vi "LinearSystemId_CreateFlywheelSystem.vi"(9 "G":dbl, 10 "jKgMetersSquared":dbl, 11 "DCMOTOR":T1 {"Jr_KgM2" format="%13.5p"; "L_H" format="%13.5p"; "Kt_NMPerAmp" format="%13.5p"; "KvINV_RadPerSecPerVolt" format="%13.5p"; "R_Ohms" format="%13.5p"; "FreeSpeed_RadPerSec" format="%13.5p"; "FreeCurrent_Amps" format="%13.5p"; "StallCurrent_Amps" format="%13.5p"; "StallTorque_NM" format="%13.5p"; "nominalVoltage_Volts" format="%13.5p"}) -> (0 "Error":bool, 3 "Linearsystem":T2)   [LabVIEW 2019, in "Trajectory_Library.lvlib"]
doc: "Create a state-space model of a flywheel system. The states of the system are [angular velocity], inputs are [voltage], and outputs are [angular velocity].\n\n\nThe flywheel linear system definition is:\n - States\n - angular velocity (Rad/Sec)\n - Inputs:\n - motor voltage\n - Outputs:\n - angular velocity (rad/sec)\n\n\nInputs: \n - motor -- The motor (or gearbox) attached to the arm.\n - jKgMetersSquared -- The moment of inertia J of the flywheel.\n - G -- The reduction between motor and drum, as a ratio of output to input.\n\nOutputs:\n - LinearSystem -- A LinearSystem representing the given characterized constants.\n - Error -- A boolean indicating an error occured creating the system. A value of TRUE indicates an error."
uses:
  Trajectory_Library.lvlib
  TypeDef/LINEAR_SYSTEM.ctl
  <vilib>/Analysis/Matrix/Datatypes/RealMatrix.ctl
  TypeDef/DCMOTOR.CTL
  MatrixHelper_CoerceSize.vi
  <vilib>/Analysis/7linalg.llb/Create Special Matrix.vi
  <vilib>/Analysis/7linalg.llb/Create Special Real Matrix.vi
  <vilib>/Analysis/Matrix/NI_Matrix.lvlib
panel:
  # "<States,States>"
  # "<States,Inputs>"
  # "<Outputs,States>"
  # "<Outputs,Inputs>"
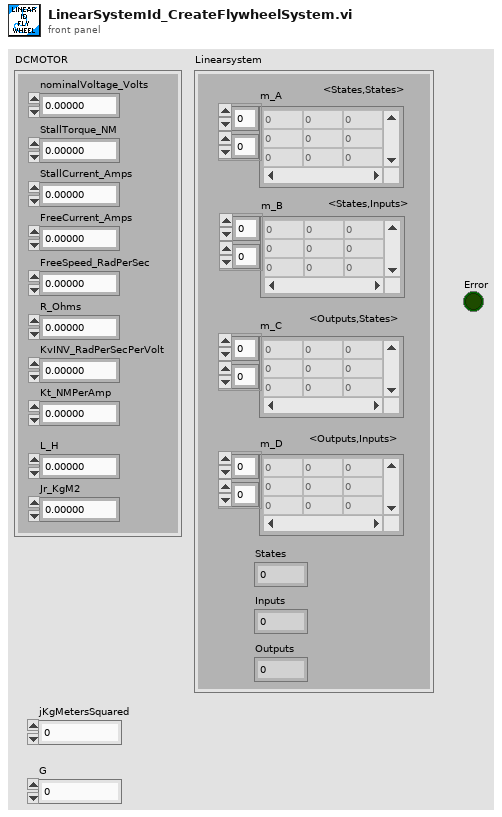
[diagram p1: front panel]
types:
  T1 = typedef "Trajectory_Library.lvlib/DCMOTOR.CTL" = cluster{"nominalVoltage_Volts":dbl, "StallTorque_NM":dbl, "StallCurrent_Amps":dbl, "FreeCurrent_Amps":dbl, "FreeSpeed_RadPerSec":dbl, "R_Ohms":dbl, "KvINV_RadPerSecPerVolt":dbl, "Kt_NMPerAmp":dbl, "L_H":dbl, "Jr_KgM2":dbl}
  T2 = typedef "Trajectory_Library.lvlib/LINEAR_SYSTEM.ctl" = cluster{"m_A":T3, "m_B":T3, "m_C":T3, "m_D":T3, "States":i32, "Inputs":i32, "Outputs":i32}
  T3 = typedef "NI_Matrix.lvlib/RealMatrix.ctl" = dbl[][]
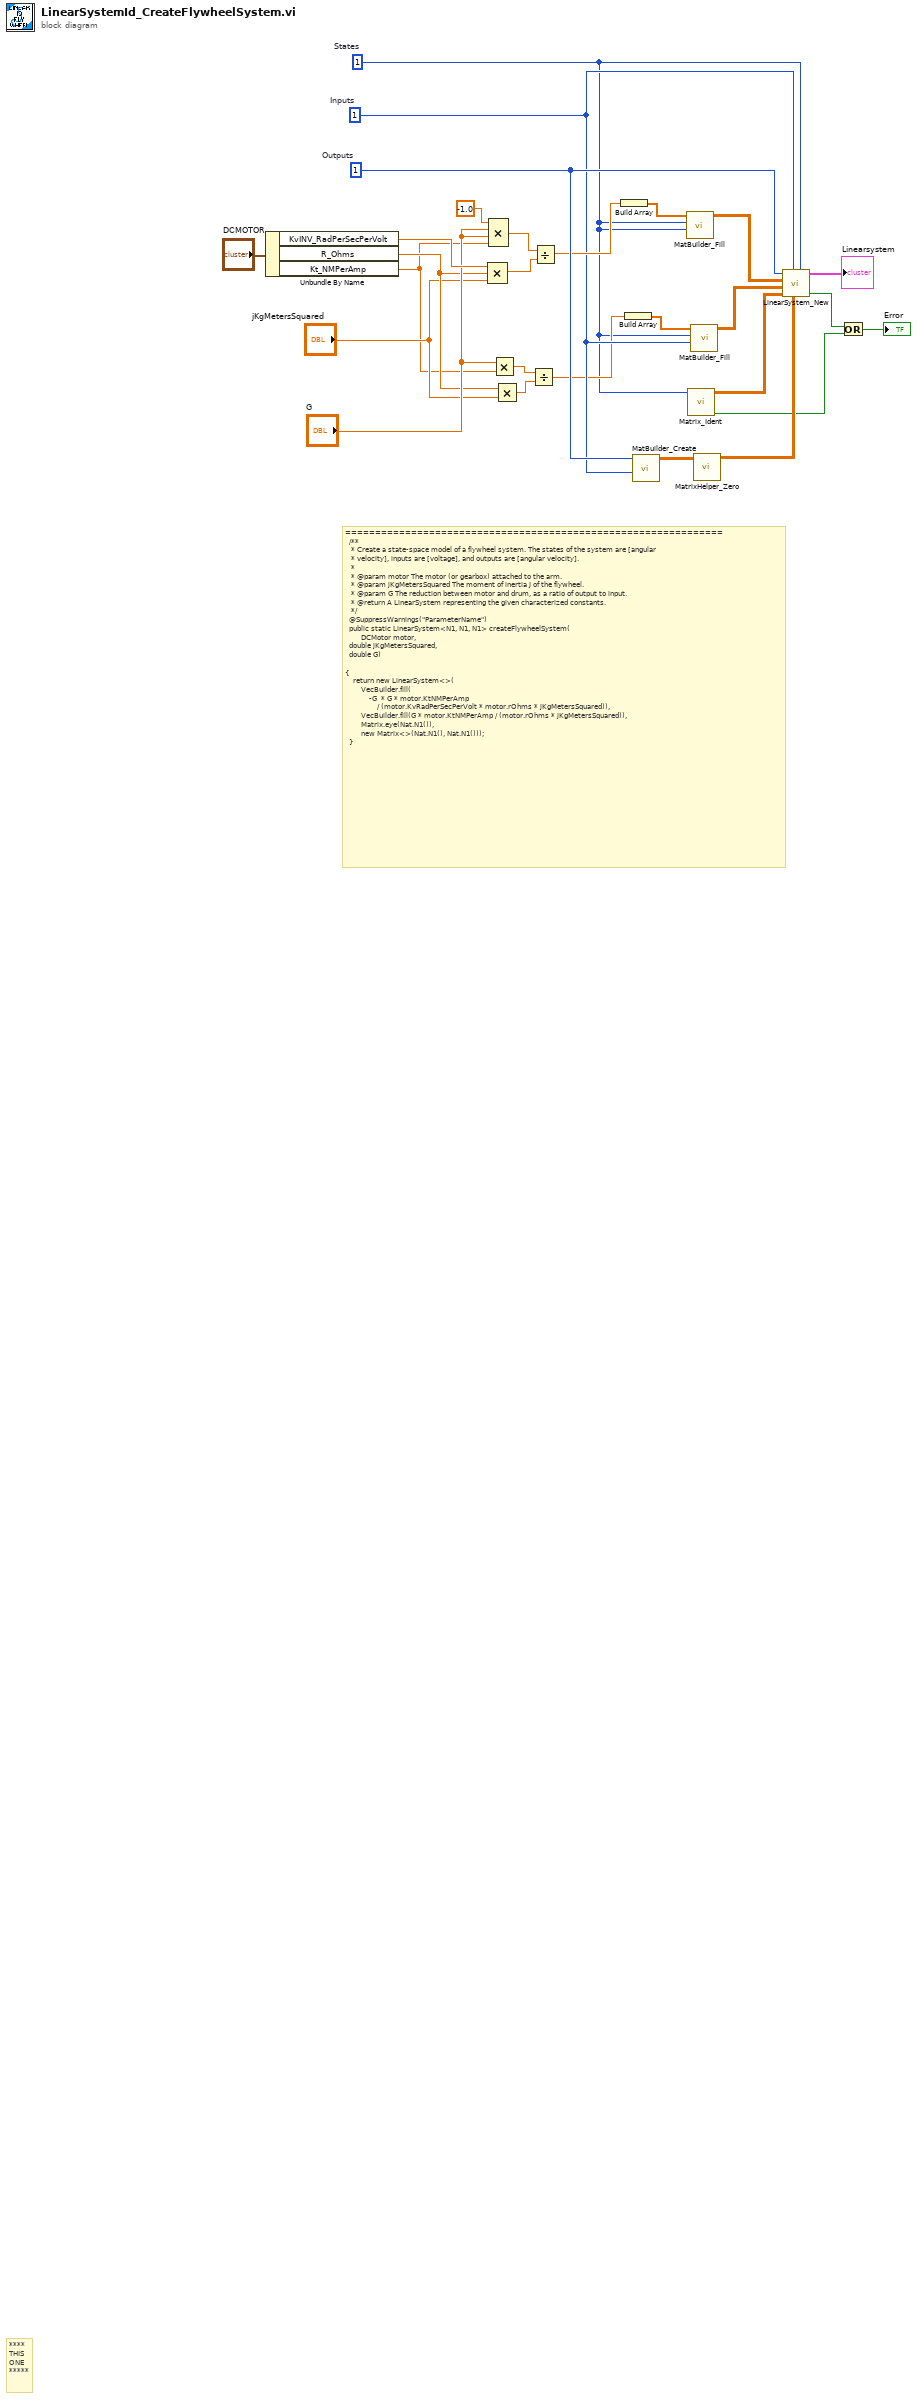
[diagram p0: block diagram]
diagram:
  w5 = 1  # States
  w8 = 1  # Inputs
  w15 = 1  # Outputs
  # "===============================================================\n  /**\n   * Create a state-space model of a flywheel system. The states of the system are [angular\n   * velocity], inputs are [voltage], and outputs are [angular velocity].\n   *\n   * @param motor The motor (or gearbox) attached to the arm.\n   * @param jKgMetersSquared The moment of inertia J of the flywheel.\n   * @param G The reduction between motor and drum, as a ratio of output to input.\n   * @return A LinearSystem representing the given characterized constants.\n   */\n  @SuppressWarnings(\"ParameterName\")\n  public static LinearSystem<N1, N1, N1> createFlywheelSystem(\n      \t\tDCMotor motor, \n\t\tdouble jKgMetersSquared, \n\t\tdouble G) \n\n{\n    return new LinearSystem<>(\n        VecBuilder.fill(\n            -G  * G * motor.KtNMPerAmp\n                / (motor.KvRadPerSecPerVolt * motor.rOhms * jKgMetersSquared)),\n        VecBuilder.fill(G * motor.KtNMPerAmp / (motor.rOhms * jKgMetersSquared)),\n        Matrix.eye(Nat.N1()),\n        new Matrix<>(Nat.N1(), Nat.N1()));\n  }"
  # "****\nTHIS\nONE\n*****"
  n1 = Unbundle By Name("DCMOTOR") -> ("KvINV_RadPerSecPerVolt"=w24:dbl, "R_Ohms"=w20:dbl, "Kt_NMPerAmp"=w16:dbl)
  n2 = Compound Arithmetic op=MULTIPLY(w24, w20, "jKgMetersSquared") -> (w22:dbl)
  n3 = Compound Arithmetic op=MULTIPLY(-1.0 ("value"), "G", "G", w16) -> (w23:dbl)
  n4 = Multiply(x="G", y=w16) -> (x*y=w18:dbl)
  n5 = Multiply(x=w20, y="jKgMetersSquared") -> (x*y=w17:dbl)
  n6 = Divide(x=w18, y=w17) -> (x/y=w7:dbl)
  n7 = Divide(x=w23, y=w22) -> (x/y=w11:dbl)
  n8 = Build Array(w11) -> (w12:dbl[])
  n9 = Build Array(w7) -> (w9:dbl[])
  n10 = call "MatBuilder_Create.vi"("Columns"=w8, "Rows"=w15) -> ("output matrix"=w14:T3)  [unwired: 9 in]
  n11 = call "MatBuilder_Fill.vi"("Columns"=w5, "Rows"=w5, "Value List"=w12) -> ("output matrix"=w10:T3)  [unwired: 8 in]
  n12 = call "Matrix_Ident.vi"("Size"=w5) -> ("Error"=w3:bool, "output matrix"=w4:T3)  [unwired: 9 in]
  n13 = call "MatBuilder_Fill.vi"("Columns"=w8, "Rows"=w5, "Value List"=w9) -> ("output matrix"=w6:T3)  [unwired: 8 in]
  n14 = call "MatrixHelper_Zero.vi"("input matrix"=w14) -> ("output matrix"=w13:T3)  [unwired: 10 in]
  n15 = call "LinearSystem_New.vi"("States"=w5, "D"=w13, "Inputs"=w8, "C"=w4, "B"=w6, "A"=w10, "Outputs"=w15) -> ("Size Coerced"=w2:bool, "Linearsystem"=→"Linearsystem":T2)  [unwired: 3 in]
  n16 = Or(x=w2, y=w3) -> (x .or. y?=→"Error":bool)
